vi "ShareVariableHandler.vi"   [LabVIEW 2026]
uses:
  Typedefs/ServoCommand.ctl
  Typedefs/BeltCtrl.ctl
  StateMachine/Globals.vi
types:
  T1 = typedef "BeltCtrl.ctl" = enum16{"Off", "Forward", "Back", "Coast", "Brake", ""}
  T2 = typedef "ServoCommand.ctl" = enum16{"colour 1", "Colour2", "Colour3", "Reject"}
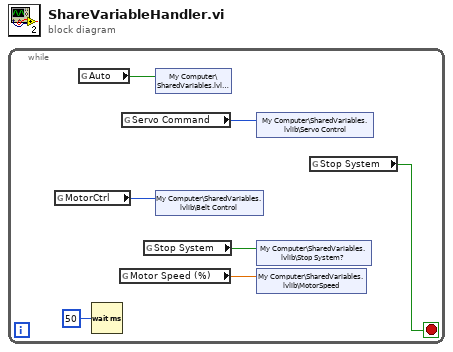
[diagram p0: block diagram]
diagram:
  n1 = while {
    stop <- w5 stop-if-true
    n2 = global read "Globals.vi" "MotorCtrl"() -> (w7:T1)
    n3 = global read "Globals.vi" "Auto"() -> (w3:bool)
    n4 = Wait (ms)(milliseconds to wait=u32 50) -> ()  [unwired: 1 out]
    n5 = global read "Globals.vi" "Motor Speed (%)"() -> (w6:dbl)
    n6 = global read "Globals.vi" "Servo Command"() -> (w4:T2)
    n7 = global read "Globals.vi" "Stop System"() -> (w2:bool)
    n8 = shared-variable "My Computer\\SharedVariables.lvlib\\Auto?"(w3) -> ()  [unwired: 1 in, 1 out]
    n9 = shared-variable "My Computer\\SharedVariables.lvlib\\Belt Control"(w7) -> ()  [unwired: 1 in, 1 out]
    n10 = shared-variable "My Computer\\SharedVariables.lvlib\\Servo Control"(w4) -> ()  [unwired: 1 in, 1 out]
    n11 = shared-variable "My Computer\\SharedVariables.lvlib\\Stop System?"(w2) -> ()  [unwired: 1 in, 1 out]
    n12 = shared-variable "My Computer\\SharedVariables.lvlib\\MotorSpeed"(w6) -> ()  [unwired: 1 in, 1 out]
    n13 = global read "Globals.vi" "Stop System"() -> (w5:bool)
  }
